vi "SPARK Close.vi"(8 "error in (no error)":errorcluster, 11 "Spark refnum":T1) -> (0 "error out":errorcluster)   [LabVIEW 2023, in "REVLibDriver.lvlib"]
uses:
  <vilib>/REVLibDriver/REVLibDriver.lvlib
  <vilib>/REV Custom Controls/REVSparkRefnum.ctl
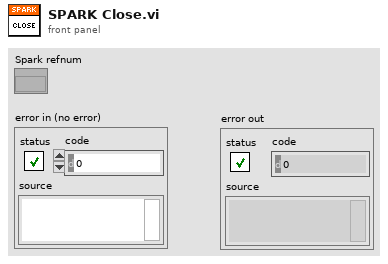
[diagram p1: front panel]
types:
  T1 = typedef "REVLibDriver.lvlib/REVSparkRefnum.ctl" = refnum<k20>
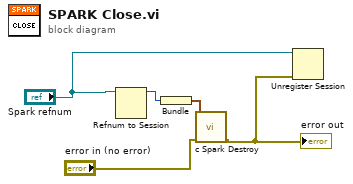
[diagram p0: block diagram]
diagram:
  n1 = Refnum to Session(7:"Spark refnum") -> (3:w3:u64)  [unwired: 1 in, 1 out]
  n2 = Bundle("Session"=w3) -> (w2:cluster{"Session":u64})  [unwired: 1 in]
  n3 = call <vilib>:"c Spark Destroy.vi"("error in (no error)"="error in (no error)", "handle"=w2) -> ("error out"=w1:errorcluster)  [unwired: 8 in, 1 out]
  "error out" <- w1
  n4 = Unregister Session(8:w1, 11:"Spark refnum") -> ()  [unwired: 1 out]
